vi "Next_Core.vi"(8 "error in (no error)":errorcluster, 10 "PGJDPResult in":refnum<class "Result.lvclass">, 11 "SqlMapper in":refnum<class "SqlMapper.lvclass">) -> (0 "error out":errorcluster, 1 "Found":bool, 2 "Row as Variant":variant, 3 "SqlMapper out":refnum<class "SqlMapper.lvclass">)   [LabVIEW 2020, in "ORM_sqlite_jdp.lvlib" / "Result.lvclass"]
uses:
  Result.lvclass
  <vilib>/Viviota/shared/ORM.lvlibp/SqlMapper/SqlMapper.lvclass
  Result.lvclass/Result.ctl
  <vilib>/drjdpowell/SQLite Library/SQL Statement/SQL Statement.lvclass/SQL Statement.ctl
  <vilib>/drjdpowell/SQLite Library/SQL Statement/Get Column Names.vi
  <vilib>/drjdpowell/SQLite Library/SQL Statement/Column Type_decl.vi
  <vilib>/drjdpowell/SQLite Library/SQL Statement/Get Column Count.vi
  <vilib>/drjdpowell/SQLite Library/SQL Statement/Write Next Column.vi
  <vilib>/drjdpowell/SQLite Library/SQL Statement/Get Column Name.vi
  <vilib>/drjdpowell/SQLite Library/SQL Statement/Column Variant.vi
  <vilib>/drjdpowell/SQLite Library/SQL Statement/Column Timestamp.vi
  <vilib>/drjdpowell/SQLite Library/SQL Statement/Error Message.vi
  <vilib>/drjdpowell/SQLite Library/SQL Statement/SQL Statement.lvclass
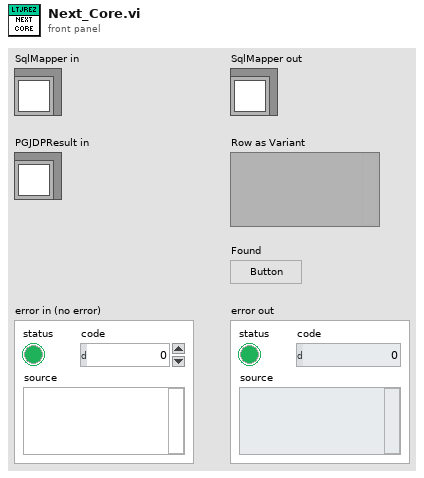
[diagram p1: front panel]
types:
  T1 = cluster{"SQL Statement":refnum<class "SQL Statement.lvclass">, "Headers":string[], "DeclaredTypes":string[]}
  T2 = cluster{"SQL Statement":refnum<class "SQL Statement.lvclass">, "Column:Column Names":string[], string[]}
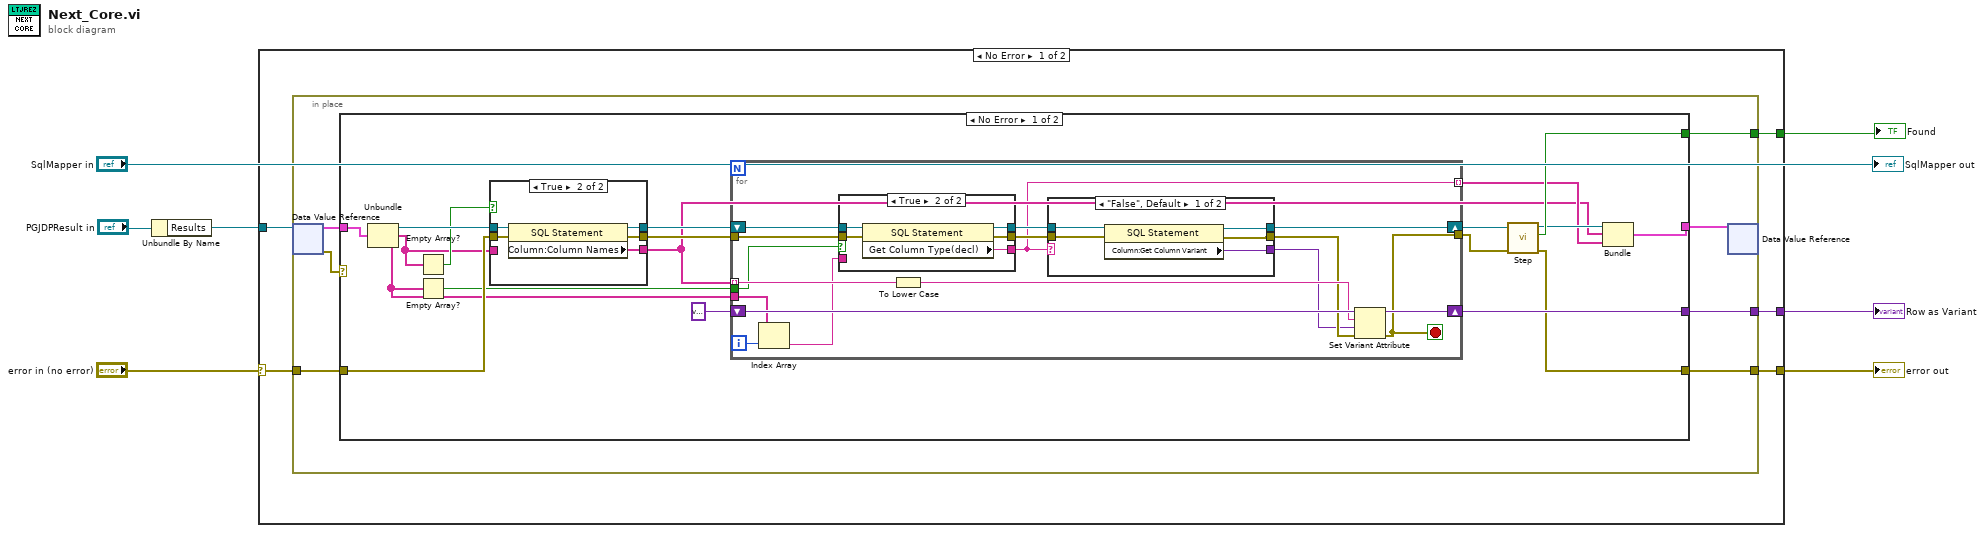
[diagram p0: block diagram]
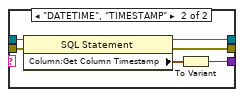
[diagram p4: hidden frame]
diagram:
  n1 = Unbundle By Name("PGJDPResult in") -> ("Results"=w2:refnum<data-value>)
  n2 = case shown="No Error" "error in (no error)" {
    selector: "error in (no error)" -> [w12 w85]
    tunnel: [w11 w85] -> w4
    tunnel: [w10 _] -> w3
    tunnel: w2 -> [w9 _]
    tunnel: [w8 _] -> w1
    frame No Error {
      n3 = in-place {
        in-place-border: w12 -> [w19]
        in-place-border: [w18] -> w11
        in-place-border: [w17] -> w10
        in-place-border: [w14] -> w8
        n4 = in-place-dvr #1(w9) -> (w16:T1, w13:errorcluster)
        n5 = case shown="No Error" w13 {
          selector: w13 -> [_ w84]
          tunnel: w19 -> [w35 _]
          tunnel: [w30 w84] -> w18
          tunnel: [w34 _] -> w17
          tunnel: w16 -> [w29 w83]
          tunnel: [w23 w83] -> w15
          tunnel: [w31 _] -> w14
          frame No Error {
            n6 = Unbundle(w29) -> ("SQL Statement"=w28:refnum<class "SQL Statement.lvclass">, "Headers"=w26:string[], "DeclaredTypes"=w24:string[])
            n7 = Empty Array?(array=w26) -> (empty?=w27:bool)
            n8 = Empty Array?(array=w24) -> (empty?=w25:bool)
            n9 = case shown="True" w27 {
              tunnel: [w41 w46] -> w38
              tunnel: [w40 w45] -> w20
              tunnel: [w39 w44] -> w36
              tunnel: w35 -> [w39 w43]
              tunnel: w28 -> [w41 w42]
              tunnel: w26 -> [w40 _]
              frame False {
              }
              frame True {
                n10 = property class="SQL Statement"(reference=w42, error in=w43) -> (reference out=w46:refnum<class "SQL Statement.lvclass">, error out=w44:errorcluster, "Column:Column Names"=w45:string[])
              }
            }
            n11 = for {
              tunnel: w20 -> [w60] mode=indexing
              shift-right: [w61] -> w34
              shift-left: variant -> [w62]
              tunnel: w36 -> [w58]
              tunnel: [w57] -> w32
              shift-right: [w53] -> w33
              shift-left: w38 -> [w63]
              tunnel: w25 -> [w51]
              tunnel: w24 -> [w48]
              tunnel: [w50] -> w21 mode=indexing
              i -> [w49]
              stop <- w57 stop-if-true
              n12 = Index Array(array=w48, index=w49) -> (element=w47:string)
              n13 = case shown="True" w51 {
                tunnel: w63 -> [w65 w71]
                tunnel: [w64 w70] -> w59
                tunnel: w58 -> [w64 w69]
                tunnel: [w65 w68] -> w54
                tunnel: [w66 w67] -> w50
                tunnel: w47 -> [w66 _]
                frame False {
                }
                frame True {
                  n14 = property class="SQL Statement"(reference=w71, error in=w69) -> (reference out=w68:refnum<class "SQL Statement.lvclass">, error out=w70:errorcluster, "Get Column Type(decl)"=w67:string)
                }
              }
              n15 = To Lower Case(string=w60) -> (all lower case string=w56:string)
              n16 = case shown="\"False\", Default" w50 {
                tunnel: w59 -> [w75 w82]
                tunnel: [w73 w81] -> w55
                tunnel: w54 -> [w76 w80]
                tunnel: [w74 w79] -> w53
                tunnel: [w72 w77] -> w52
                frame "False", Default {
                  n17 = property class="SQL Statement"(reference=w76, error in=w75) -> (reference out=w74:refnum<class "SQL Statement.lvclass">, error out=w73:errorcluster, "Column:Get Column Variant"=w72:variant)
                }
                frame "DATETIME", "TIMESTAMP" {
                  n18 = property class="SQL Statement"(reference=w80, error in=w82) -> (reference out=w79:refnum<class "SQL Statement.lvclass">, error out=w81:errorcluster, "Column:Get Column Timestamp"=w78:timestamp)
                  n19 = To Variant(anything=w78) -> (Variant=w77:variant)
                }
              }
              n20 = Set Variant Attribute(Variant=w62, name=w56, value=w52, error in=w55) -> (Variant out=w61:variant, error out=w57:errorcluster)  [unwired: 1 out]
            }
            n21 = call <vilib>:"Step.vi"("error in (no error)"=w32, "SQL Statement in"=w33) -> ("error out"=w30:errorcluster, "Row returned"=w31:bool, "SQL Statement"=w22:refnum<class "SQL Statement.lvclass">)  [unwired: 7 in]
            n22 = Bundle("SQL Statement"=w22, "Column:Column Names"=w20, w21) -> (w23:T2)  [unwired: 1 in]
          }
          frame Error {
          }
        }
        n23 = in-place-dvr #1(w15) -> ()  [unwired: 2 out]
      }
    }
    frame Error {
    }
  }
  "error out" <- w4
  "Row as Variant" <- w3
  "Found" <- w1
  "SqlMapper out" <- "SqlMapper in"
